vi "XPN Get Wrapper Version.vi"(8 "error in (no error)":errorcluster) -> (0 "error out":errorcluster, 3 "function return":string)   [LabVIEW 2025, in "xPanelWrapper.lvlib"]
doc: "XPN_API const char* XPN_GetWrapperVersion();"
uses:
  xPanelWrapper.lvlib
  xPanelWrapper.dll
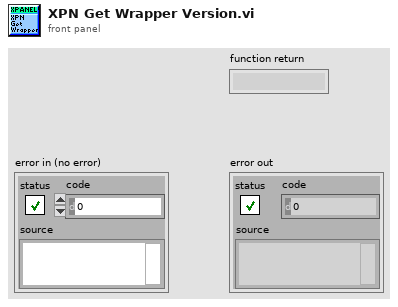
[diagram p1: front panel]
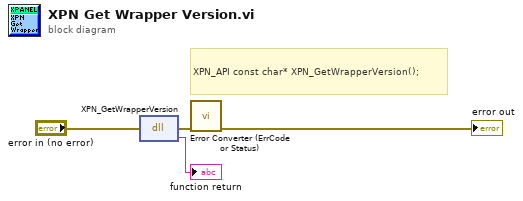
[diagram p0: block diagram]
diagram:
  # "XPN_API const char* XPN_GetWrapperVersion();"
  n1 = dll-call lib="E:/GitHub/xPanelWrapper/xPanelWrapperLvLib/xPanelWrapper.*" fn="XPN_GetWrapperVersion"(error in="error in (no error)") -> (error out=w2:errorcluster, →"function return":string)  [unwired: 2 in, 1 out]
  n2 = call "Error Converter (ErrCode or Status).vi"("error in (no error)"=w2) -> ("error out"=→"error out":errorcluster)  [unwired: 10 in]
